vi "laser_calibrate.vi"(10 "Laser Active":bool, 11 "Calibration Mode":enum32{"Manual", "Automatic"}(tab)=enum."Automatic") -> ()   [LabVIEW 2025, in "tSNIP.lvlib"]
uses:
  tSNIP.lvlib
panel:
  out "Measured Power":cluster{"Value":dbl, "Units":dbl}={"Value"=0.0, "Units"=0.001} {"Units" items=["mW"=0.001, "W"=1.0]; "Value" min=0.0 step=50.0}
  out "Power Out":cluster{"Value":dbl, "Units":dbl}={"Value"=0.0, "Units"=0.001} {"Units" items=["mW"=0.001, "W"=1.0]; "Value" min=0.0 step=50.0}
  out "Current Out":cluster{"Value":dbl, "Units":dbl}={"Value"=0.0, "Units"=0.001} {"Units" items=["mA"=0.001, "A"=1.0]; "Value" min=0.0 step=50.0}
  in  "Current":cluster{"Value":dbl, "Units":dbl}={"Value"=0.0, "Units"=0.001} {"Units" items=["mA"=0.001, "A"=1.0]; "Value" min=0.0 step=50.0}
  in  "Config file path":path=path "C:/Users/TDT/Box/Electrical Nerve Block Institute/Software/LabVIEW/tSNIP/calibration_config.csv"
  in  "Exit":bool
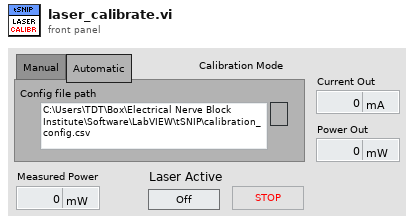
[diagram p1: front panel]
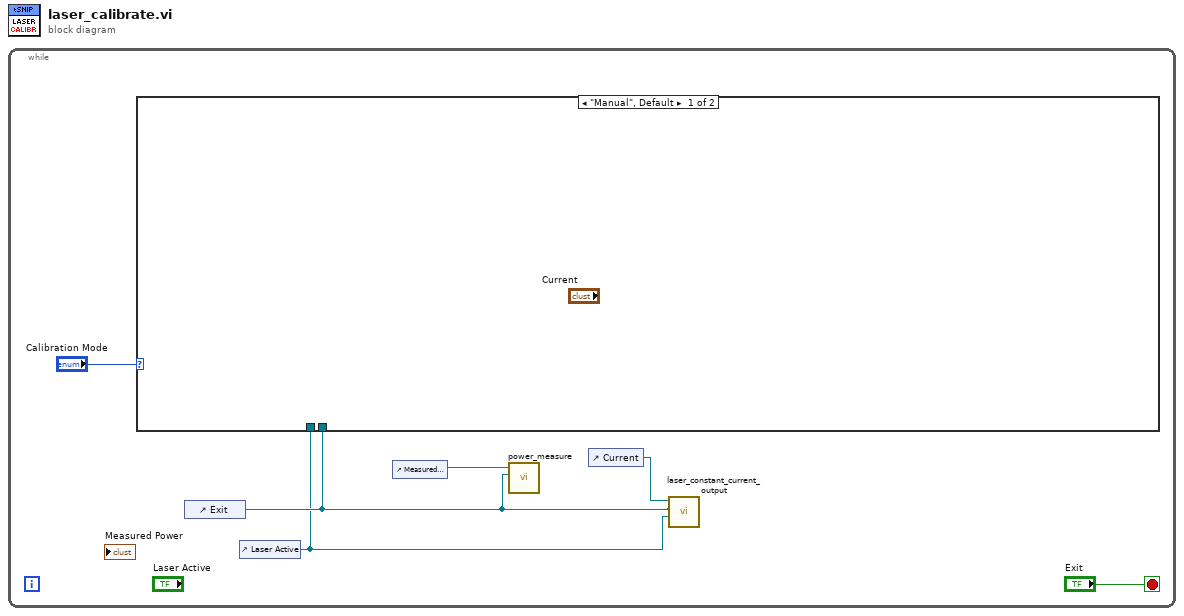
[diagram p0: block diagram]
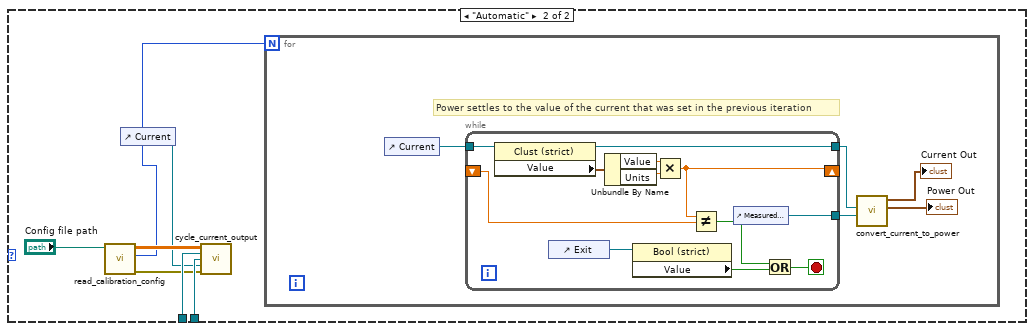
[diagram p2: hidden frame]
diagram:
  n1 = while {
    stop <- "Exit" stop-if-true
    n2 = control-ref of="Exit"() -> (w4:refnum<vi>)
    n3 = control-ref of="Laser Active"() -> (w3:refnum<vi>)
    n4 = case shown="\"Manual\", Default" "Calibration Mode" {
      tunnel: w4 -> [_ w11]
      tunnel: w3 -> [_ w10]
      frame "Manual", Default {
      }
      frame "Automatic" {
        n5 = call "read_calibration_config.vi"("Config file path"="Config file path") -> ("error out"=w7:errorcluster, "Num Points"=w8:i32, "Config Parameters"=w12:dbl[][])  [unwired: 8 in]
        n6 = control-ref of="Current"() -> (w9:refnum<vi>)
        n7 = call "cycle_current_output.vi"("Config Parameters"=w12, "Laser Active Ref"=w10, "Stop Ref"=w11, "Current Ref"=w9, "error in"=w7) -> ()  [unwired: 10 in, 1 out]
        n8 = for {
          N: w8 -> [_]
          # "Power settles to the value of the current that was set in the previous iteration"
          n9 = control-ref of="Current"() -> (w14:refnum<vi>)
          n10 = while {
            shift-right: [w27] -> _
            shift-left: _ -> [w26]
            tunnel: [w25] -> w16
            tunnel: [w19] -> w15
            tunnel: w14 -> [w20]
            stop <- w21 stop-if-true
            n11 = property class="Clust (strict)"(reference=w20) -> (reference out=w25:refnum<vi>, "Value"=w30:cluster{"Value":dbl, "Units":dbl})  [unwired: 1 in, 1 out]
            n12 = control-ref of="Exit"() -> (w23:refnum<vi>)
            n13 = Unbundle By Name(w30) -> ("Value"=w29:dbl, "Units"=w28:dbl)
            n14 = property class="Bool (strict)"(reference=w23) -> ("Value"=w22:bool)  [unwired: 1 in, 2 out]
            n15 = Multiply(x=w29, y=w28) -> (x*y=w27:dbl)
            n16 = Not Equal?(x=w27, y=w26) -> (x != y?=w24:bool)
            n17 = control-ref of="Measured Power"() -> (w19:refnum<vi>)
            n18 = Or(x=w24, y=w22) -> (x .or. y?=w21:bool)
          }
          n19 = call "convert_current_to_power.vi"("Measured Power Refnum"=w15, "Current Ref"=w16) -> ("Power Out"=→"Power Out":cluster{"Value":dbl, "Units":dbl}, "Current Out"=→"Current Out":cluster{"Value":dbl, "Units":dbl})  [unwired: 8 in]
        }
      }
    }
    n20 = control-ref of="Measured Power"() -> (w1:refnum<vi>)
    n21 = call "power_measure.vi"("Stop Refnum"=w4, "Measured Power Refnum"=w1) -> ()  [unwired: 10 in]
    n22 = control-ref of="Current"() -> (w2:refnum<vi>)
    n23 = call "laser_constant_current_output.vi"("Laser Active Ref"=w3, "Stop Ref"=w4, "Current Ref"=w2) -> ()  [unwired: 9 in]
  }
